vi "update sync UI.vi"(8 "error in (no error)":errorcluster, 9 "sync ui refs":T1, 10 "engine in":refnum<class "Engine Parent Editor Node.lvclass">, 11 "shared memory editor node in":refnum<class "module editor node.lvclass">) -> (0 "error out":errorcluster, 2 "engine out":refnum<class "Engine Parent Editor Node.lvclass">, 3 "shared memory editor node out":refnum<class "module editor node.lvclass">)   [LabVIEW 2014, in "Shared Memory editor node.lvclass"]
uses:
  Shared Memory editor node.lvclass
  <vilib>/NI/DCAF/Tag Editor Core/Configuration Editor/Classes/Module editor node/module editor node.lvclass
  ui controls sync.ctl
  <vilib>/NI/DCAF/Tag Editor Core/Configuration Editor/Classes/Engine Parent/Engine Parent Editor Node.lvclass
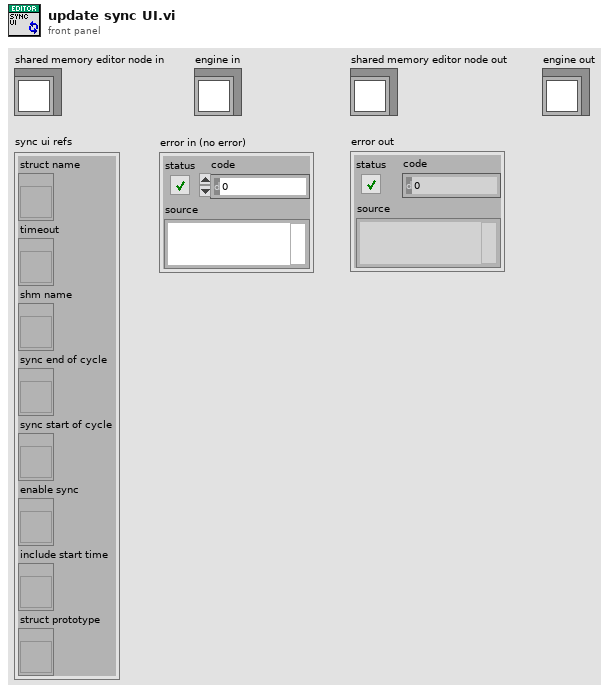
[diagram p1: front panel]
types:
  T1 = typedef "Shared Memory editor node.lvclass/ui controls sync.ctl" = cluster{"struct name":refnum<vi>, "timeout":refnum<vi>, "shm name":refnum<vi>, "sync end of cycle":refnum<vi>, "sync start of cycle":refnum<vi>, "enable sync":refnum<vi>, "include start time":refnum<vi>, "struct prototype":refnum<vi>}
  T2 = typedef "Shared Memory configuration.lvclass/sync item.ctl" = cluster{"mechanism":T3, "name":string}
  T3 = typedef "Shared Memory configuration.lvclass/sync mechanism.ctl" = enum16{"Semaphore"}
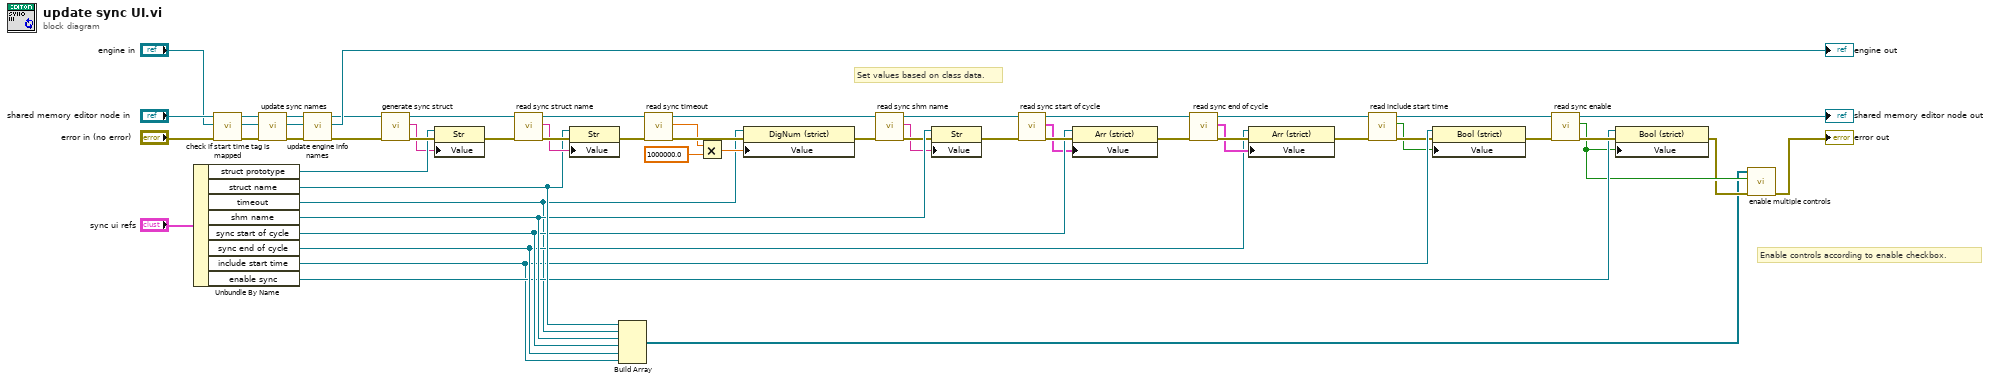
[diagram p0: block diagram]
diagram:
  # "Enable controls according to enable checkbox."
  # "Set values based on class data."
  n1 = Unbundle By Name("sync ui refs") -> ("struct prototype"=w12:refnum<vi>, "struct name"=w46:refnum<vi>, "timeout"=w25:refnum<vi>, "shm name"=w45:refnum<vi>, "sync start of cycle"=w39:refnum<vi>, "sync end of cycle"=w33:refnum<vi>, "include start time"=w23:refnum<vi>, "enable sync"=w31:refnum<vi>)
  n2 = call "check if start time tag is mapped.vi"("error in"="error in (no error)", "engine in"="engine in", "shared memory editor node in"="shared memory editor node in") -> ("error out"=w9:errorcluster, "engine out"=w7:refnum<class "Engine Parent Editor Node.lvclass">, "shared memory editor node out"=w8:refnum<class "module editor node.lvclass">)  [unwired: 5 in, 1 out]
  n3 = call "update sync names.vi"("error in"=w9, "engine in"=w7, "shared memory editor node in"=w8) -> ("error out"=w6:errorcluster, "engine out"=w5:refnum<class "Engine Parent Editor Node.lvclass">, "shared memory editor node out"=w4:refnum<class "module editor node.lvclass">)  [unwired: 6 in]
  n4 = call "update engine info names.vi"("error in"=w6, "engine in"=w5, "shared memory editor node in"=w4) -> ("error out"=w3:errorcluster, "engine out"=→"engine out":refnum<class "Engine Parent Editor Node.lvclass">, "shared memory editor node out"=w1:refnum<class "module editor node.lvclass">)  [unwired: 6 in]
  n5 = call "generate sync struct.vi"("error in (no error)"=w3, "shared memory editor node in"=w1) -> ("error out"=w14:errorcluster, "struct string"=w11:string, "shared memory editor node out"=w10:refnum<class "module editor node.lvclass">)  [unwired: 7 in]
  n6 = property class="Str"(reference=w12, error in=w14, "Value"=w11) -> (error out=w13:errorcluster)  [unwired: 1 out]
  n7 = call "read sync struct name.vi"("error in"=w13, "shared memory editor node"=w10) -> ("error out"=w56:errorcluster, "sync struct name"=w55:string, "shared memory editor node out"=w54:refnum<class "module editor node.lvclass">)  [unwired: 7 in]
  n8 = property class="Str"(reference=w46, error in=w56, "Value"=w55) -> (error out=w53:errorcluster)  [unwired: 1 out]
  n9 = Build Array(w46, w25, w45, w39, w33, w23) -> (w26:refnum<vi>[])
  n10 = call "read sync timeout.vi"("error in"=w53, "shared memory editor node"=w54) -> ("error out"=w50:errorcluster, "sync struct name"=w48:dbl, "shared memory editor node out"=w49:refnum<class "module editor node.lvclass">)  [unwired: 7 in]
  n11 = Multiply(x=w48, y=1000000.0) -> (x*y=w51:dbl)
  n12 = property class="DigNum (strict)"(reference=w25, error in=w50, "Value"=w51) -> (error out=w47:errorcluster)  [unwired: 1 out]
  n13 = call "read sync shm name.vi"("error in"=w47, "shared memory editor node"=w49) -> ("error out"=w44:errorcluster, "shm name"=w43:string, "shared memory editor node out"=w42:refnum<class "module editor node.lvclass">)  [unwired: 7 in]
  n14 = property class="Str"(reference=w45, error in=w44, "Value"=w43) -> (error out=w41:errorcluster)  [unwired: 1 out]
  n15 = call "read sync start of cycle.vi"("error in"=w41, "shared memory editor node"=w42) -> ("error out"=w40:errorcluster, "sync start of cycle"=w38:T2[], "shared memory editor node out"=w37:refnum<class "module editor node.lvclass">)  [unwired: 7 in]
  n16 = property class="Arr (strict)"(reference=w39, error in=w40, "Value"=w38) -> (error out=w36:errorcluster)  [unwired: 1 out]
  n17 = call "read sync end of cycle.vi"("error in"=w36, "shared memory editor node"=w37) -> ("error out"=w35:errorcluster, "sync end of cycle"=w34:T2[], "shared memory editor node out"=w21:refnum<class "module editor node.lvclass">)  [unwired: 7 in]
  n18 = property class="Arr (strict)"(reference=w33, error in=w35, "Value"=w34) -> (error out=w22:errorcluster)  [unwired: 1 out]
  n19 = call "read include start time.vi"("error in"=w22, "shared memory editor node"=w21) -> ("error out"=w19:errorcluster, "include start time"=w18:bool, "shared memory editor node out"=w20:refnum<class "module editor node.lvclass">)  [unwired: 7 in]
  n20 = property class="Bool (strict)"(reference=w23, error in=w19, "Value"=w18) -> (error out=w24:errorcluster)  [unwired: 1 out]
  n21 = call "read sync enable.vi"("error in"=w24, "shared memory editor node"=w20) -> ("error out"=w32:errorcluster, "sync enable"=w30:bool, "shared memory editor node out"=→"shared memory editor node out":refnum<class "module editor node.lvclass">)  [unwired: 7 in]
  n22 = property class="Bool (strict)"(reference=w31, error in=w32, "Value"=w30) -> (error out=w29:errorcluster)  [unwired: 1 out]
  n23 = call "enable multiple controls.vi"("error in (no error)"=w29, "enabled? (T)"=w30, "controls in"=w26) -> ("error out"=→"error out":errorcluster)  [unwired: 6 in, 2 out]
